vi "VIH Utility - STR - Remove Empty Strings from 1D Array.vi"(8 "error in":errorcluster, 11 "String array in":string[](array[string])) -> (0 "error out":errorcluster, 3 "String array out":string[](array[string]))   [LabVIEW 2014]
doc: "::: VI Helpeks :::\nCopyright (c) 2000-2026 Konstantin Shifershteyn. All rights reserved."
panel:
  # "VI Helpeks\nCopyright (c) 2012-2026 Konstantin Shifershteyn"
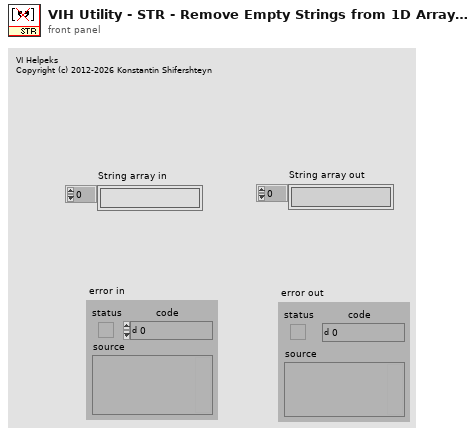
[diagram p1: front panel]
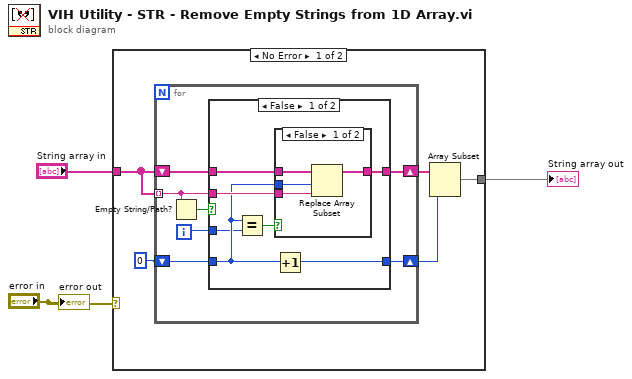
[diagram p0: block diagram]
diagram:
  n1 = case shown="No Error" "error in" {
    tunnel: "String array in" -> [w8 w30]
    tunnel: [w4 w30] -> w2
    frame No Error {
      n2 = for {
        shift-right: [w11] -> w6
        shift-left: w8 -> [w14]
        tunnel: w8 -> [w10] mode=indexing
        shift-right: [w12] -> w5
        shift-left: 0 -> [w13]
        i -> [w9]
        n3 = Empty String/Path?(string/path=w10) -> (empty?=w15:bool)
        n4 = case shown="False" w15 {
          tunnel: w14 -> [w21 w28]
          tunnel: w13 -> [w17 w29]
          tunnel: [w18 w29] -> w12
          tunnel: [w20 w28] -> w11
          tunnel: w10 -> [w19 _]
          tunnel: w9 -> [w16 _]
          frame False {
            n5 = Equal?(x=w17, y=w16) -> (x = y?=w22:bool)
            n6 = case shown="False" w22 {
              tunnel: w21 -> [w26 w27]
              tunnel: [w25 w27] -> w20
              tunnel: w19 -> [w24 _]
              tunnel: w17 -> [w23 _]
              frame False {
                n7 = Replace Array Subset(array=w26, new element=w24, index=w23) -> (w25:string[])
              }
              frame True {
              }
            }
            n8 = Increment(x=w17) -> (x+1=w18:i32)
          }
          frame True {
          }
        }
      }
      n9 = Array Subset(array=w6, length=w5) -> (w4:string[])  [unwired: 1 in]
    }
    frame Error {
    }
  }
  "String array out" <- w2
  "error out" <- "error in"
